vi "Read Batch OD By Array Index - i32.vi"(8 "error in (no error)":errorcluster, 10 "array index":i32, 11 "OD Batch in":refnum<class "OD Batch.lvclass">) -> (0 "error out":errorcluster, 2 "value":i32, 3 "OD Batch out":refnum<class "OD Batch.lvclass">)   [LabVIEW 2023, in "xnet_canopen.lvlib" / "OD Batch.lvclass"]
uses:
  OD Batch.lvclass
  OD Batch.lvclass/OD Batch.ctl
  xnet_canopen.lvlib
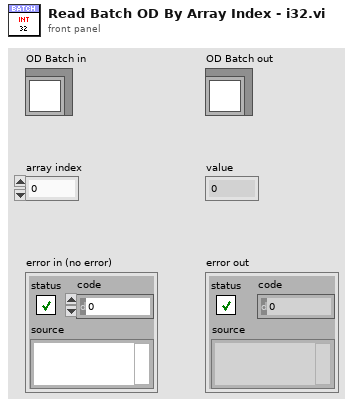
[diagram p1: front panel]
types:
  T1 = typedef "xnet_canopen.lvlib/od entry.ctl" = cluster{"OD Index":T2, "CANOpen Types":T3, "Size":u32, "Offset":u32, "Value":variant, "Initialized":bool}
  T2 = typedef "xnet_canopen.lvlib/od index.ctl" = cluster{"Index":u16, "SubIndex":u8}
  T3 = typedef "xnet_canopen.lvlib/canopen types.ctl" = u32
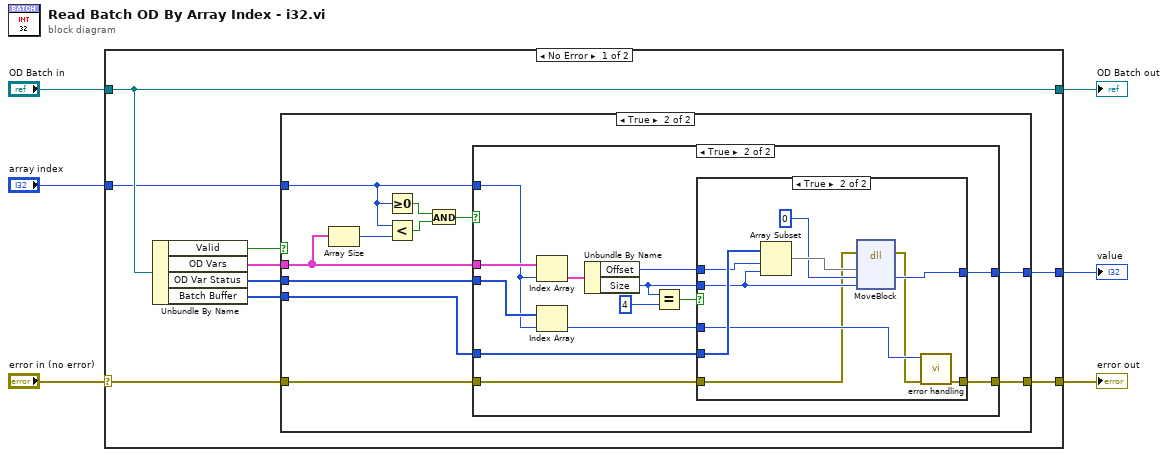
[diagram p0: block diagram]
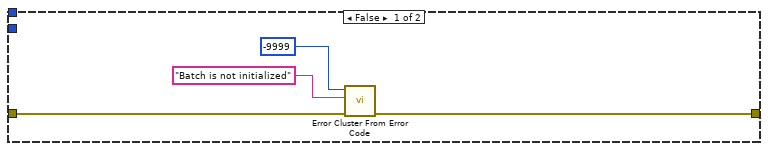
[diagram p2: hidden frame]
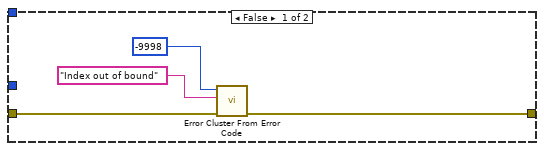
[diagram p3: hidden frame]
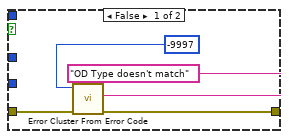
[diagram p4: hidden frame]
diagram:
  n1 = case shown="No Error" "error in (no error)" {
    selector: "error in (no error)" -> [w15 w63]
    tunnel: [w13 w63] -> w5
    tunnel: [w14 w62] -> w3
    tunnel: "OD Batch in" -> [w14 w62]
    tunnel: "array index" -> [w10 _]
    tunnel: [w7 _] -> w1
    frame No Error {
      n2 = Unbundle By Name(w14) -> ("Valid"=w12:bool, "OD Vars"=w11:T1[], "OD Var Status"=w9:i32[], "Batch Buffer"=w8:u8[])
      n3 = case shown="True" w12 {
        tunnel: w15 -> [w19 w23]
        tunnel: [w18 w22] -> w13
        tunnel: w11 -> [_ w29]
        tunnel: w10 -> [_ w27]
        tunnel: w9 -> [_ w30]
        tunnel: w8 -> [_ w21]
        tunnel: [_ w20] -> w7
        frame False {
          n4 = call <vilib>:"Error Cluster From Error Code.vi"("error in (no error)"=w19, "error message (\"\")"="Batch is not initialized" ("error message (\"\")"), "error code (0)"=-9999) -> ("error out"=w18:errorcluster)  [unwired: 6 in]
        }
        frame True {
          n5 = Array Size(array=w29) -> (size(s)=w28:i32)
          n6 = Greater Or Equal To 0?(x=w27) -> (x >= 0?=w25:bool)
          n7 = Less?(x=w27, y=w28) -> (x < y?=w26:bool)
          n8 = And(x=w25, y=w26) -> (x .and. y?=w24:bool)
          n9 = case shown="True" w24 {
            tunnel: w30 -> [_ w47]
            tunnel: w29 -> [_ w46]
            tunnel: w27 -> [_ w45]
            tunnel: w23 -> [w32 w41]
            tunnel: [w31 w40] -> w22
            tunnel: w21 -> [_ w39]
            tunnel: [_ w36] -> w20
            frame False {
              n10 = call <vilib>:"Error Cluster From Error Code.vi"("error in (no error)"=w32, "error message (\"\")"="Index out of bound" ("error message (\"\")"), "error code (0)"=-9998) -> ("error out"=w31:errorcluster)  [unwired: 6 in]
            }
            frame True {
              n11 = Index Array(array=w46, index=w45) -> (element=w44:T1)
              n12 = Index Array(array=w47, index=w45) -> (element=w35:i32)
              n13 = Unbundle By Name(w44) -> ("Offset"=w38:u32, "Size"=w37:u32)
              n14 = Equal?(x=w37, y=u32 4) -> (x = y?=w42:bool)
              n15 = case shown="True" w42 {
                tunnel: w41 -> [w49 w53]
                tunnel: [w48 w59] -> w40
                tunnel: w39 -> [_ w61]
                tunnel: w38 -> [_ w60]
                tunnel: w37 -> [_ w54]
                tunnel: [_ w56] -> w36
                tunnel: w35 -> [_ w58]
                frame False {
                  n16 = call <vilib>:"Error Cluster From Error Code.vi"("error in (no error)"=w49, "error message (\"\")"="OD Type doesn't match" ("error message (\"\")"), "error code (0)"=-9997) -> ("error out"=w48:errorcluster)  [unwired: 6 in]
                }
                frame True {
                  n17 = Array Subset(array=w61, index=w60, length=w54) -> (w57:u8[])
                  n18 = dll-call lib="LabVIEW" fn="MoveBlock"(error in=w53, "src"=w57, 0, "sz"=w54) -> (error out=w52:errorcluster, w56:i32)  [unwired: 5 in, 1 out]
                  n19 = call "error handling.vi"("error in (no error)"=w52, "return val"=w58) -> ("error out"=w59:errorcluster)  [unwired: 9 in]
                }
              }
            }
          }
        }
      }
    }
    frame Error {
    }
  }
  "error out" <- w5
  "OD Batch out" <- w3
  "value" <- w1
